vi "Read Analog Input.vi"(8 "error in (no error)":errorcluster, 11 "Devices.DAQ Device":T2) -> (0 "error out":errorcluster, 2 "Analog Input Cluster":T1, 3 "Scaled Analog Input":dbl[](array[numeric]))   [LabVIEW 2021]
uses:
  DAQNav Cluster.ctl
  Analog Cluster.ctl
  <userlib>/DAQNavi Polymorphic VI/read/DAQNavi Read (Analog 2D DBL NChan NSamp).vi
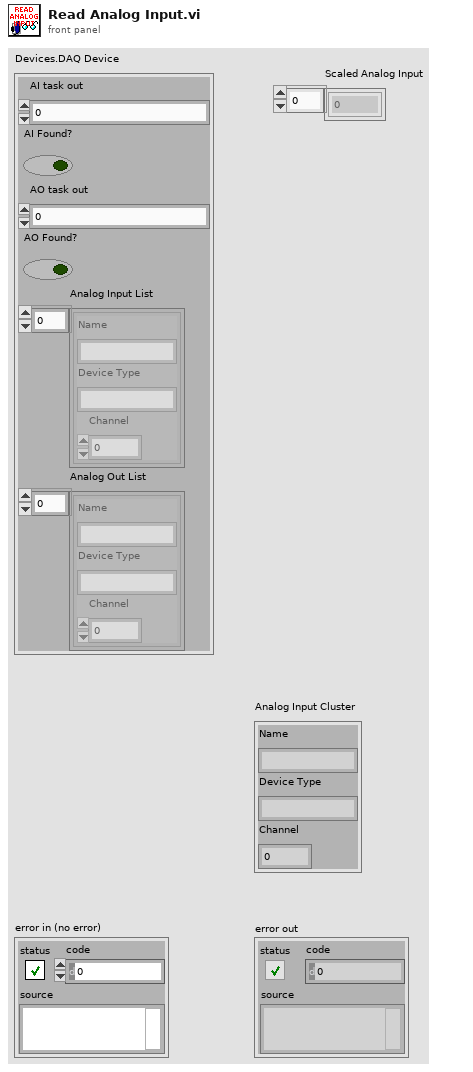
[diagram p1: front panel]
types:
  T1 = typedef "Analog Cluster.ctl" = cluster{"Name":string, "Device Type":string, "Channel":i32}
  T2 = typedef "DAQNav Cluster.ctl" = cluster{"AI task out":i32, "AI Found?":bool, "AO task out":i32, "AO Found?":bool, "Analog Input List":T1[], "Analog Out List":T1[]}
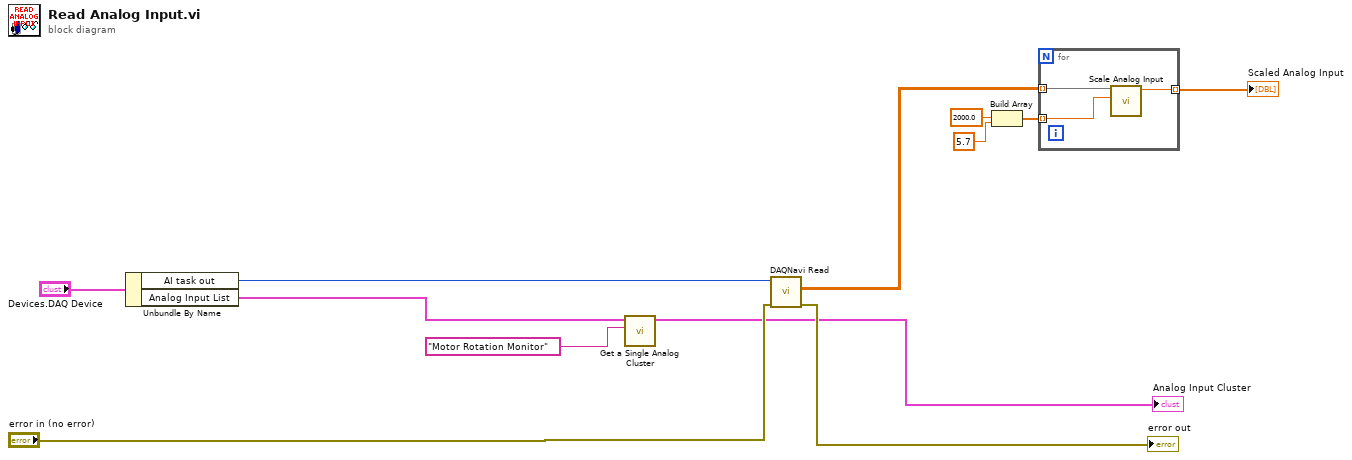
[diagram p0: block diagram]
diagram:
  n1 = Unbundle By Name("Devices.DAQ Device") -> ("AI task out"=w10:i32, "Analog Input List"=w8:T1[])
  n2 = call "Get a Single Analog Cluster.vi"("Parameter Name"="Motor Rotation Monitor", "Analog Input List"=w8) -> ("Analog Input Cluster"=→"Analog Input Cluster":T1)  [unwired: 9 in]
  n3 = call-poly <userlib>:"DAQNavi Read.vi"("error in (no error)"="error in (no error)", "task in"=w10) -> ("error out"=→"error out":errorcluster, "data"=w6:dbl[][])  [unwired: 6 in, 2 out]
  n4 = Build Array(2000.0 ("y"), 5.7 ("y")) -> (w3:dbl[])
  n5 = for {
    tunnel: w6 -> [w15] mode=indexing
    tunnel: w3 -> [w14] mode=indexing
    tunnel: [w13] -> w2 mode=indexing
    n6 = call "Scale Analog Input.vi"("y"=w14, "raw samples"=w15) -> ("Numeric"=w13:dbl)  [unwired: 9 in]
  }
  "Scaled Analog Input" <- w2
